vi "project 1.vi"() -> ()   [LabVIEW 2020]
uses:
  <vilib>/MakerHub/LINX/Public/Peripherals/Analog/Analog Read 1 Chan.vi
  <vilib>/MakerHub/LINX/Public/Peripherals/Analog/Analog Read N Chans.vi
  <vilib>/MakerHub/LINX/Private/Local IO/LinxAnalogRead.vi
  <vilib>/MakerHub/LINX/Public/Utilities/Check Channel.vi
  <vilib>/MakerHub/LINX/Public/Utilities/Open Serial.vi
  <vilib>/MakerHub/LINX/Public/Sensors/Motion/Servo/Servo Open One Channel.vi
  <vilib>/MakerHub/LINX/Private/Utilties/Generate Error.vi
  <vilib>/MakerHub/LINX/Public/Sensors/Motion/Servo/Servo Set Pulse Width One Channel.vi
  <vilib>/MakerHub/LINX/Public/Sensors/Motion/Servo/Servo Close One Channel.vi
  <vilib>/MakerHub/LINX/LMH-LINX.lvlib
  <vilib>/MakerHub/LINX/Public/Sensors/Motion/Servo/Servo.lvlib
panel:
  out "Angle":dbl=2.197357822357816
  out "Pulse width\nx+y":dbl=1024.4140625
  in  "stop":bool
  out "dv":dbl=0.1220703125
  out "Voltage 2":dbl=0.2099609375
  out "Voltage":dbl=0.33203125
  in  "Gain":dbl=200.0
  in  "Serial Port":refnum<visa-resource-name>="COM3"
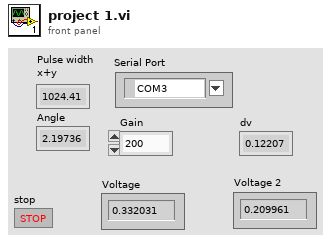
[diagram p1: front panel]
types:
  T1 = typedef "LMH-LINX.lvlib/LINX Ref.ctl" = cluster{"IO":T2, "Interface":T3, "LINX Device Config":T4}
  T2 = typedef "LMH-LINX.lvlib/Platform.ctl" = enum16{"Remote", "Local"}
  T3 = typedef "LMH-LINX.lvlib/Interface.ctl" = enum16{"Serial", "TCP"}
  T4 = typedef "LMH-LINX.lvlib/Device.lvlib/LINX Device Config.ctl" = cluster{"Interface":T3, "COM Port":refnum<visa-resource-name>, "TCP Configuration":T5, "Device Family":u8, "Device ID":u8, "Device Name":string, "TCP Ref":refnum<k5>, "Channels":T6}
  T5 = typedef "LMH-LINX.lvlib/Device.lvlib/TCP Config.ctl" = cluster{"IP Address":string, "Port":u16}
  T6 = typedef "LMH-LINX.lvlib/Channels.ctl" = cluster{"DI":u8[], "DO":u8[], "AI":u8[], "AO":u8[], "PWM":u8[], "QE":u8[], "UART":u8[], "I2C 2":u8[], "SPI":u8[], "CAN":u8[], "Servo":u8[], "AI Ref (V)":dbl, "AI Resolution (Bits)":u8, "AO Ref (V)":dbl, "AO Resolution (Bits)":u8}
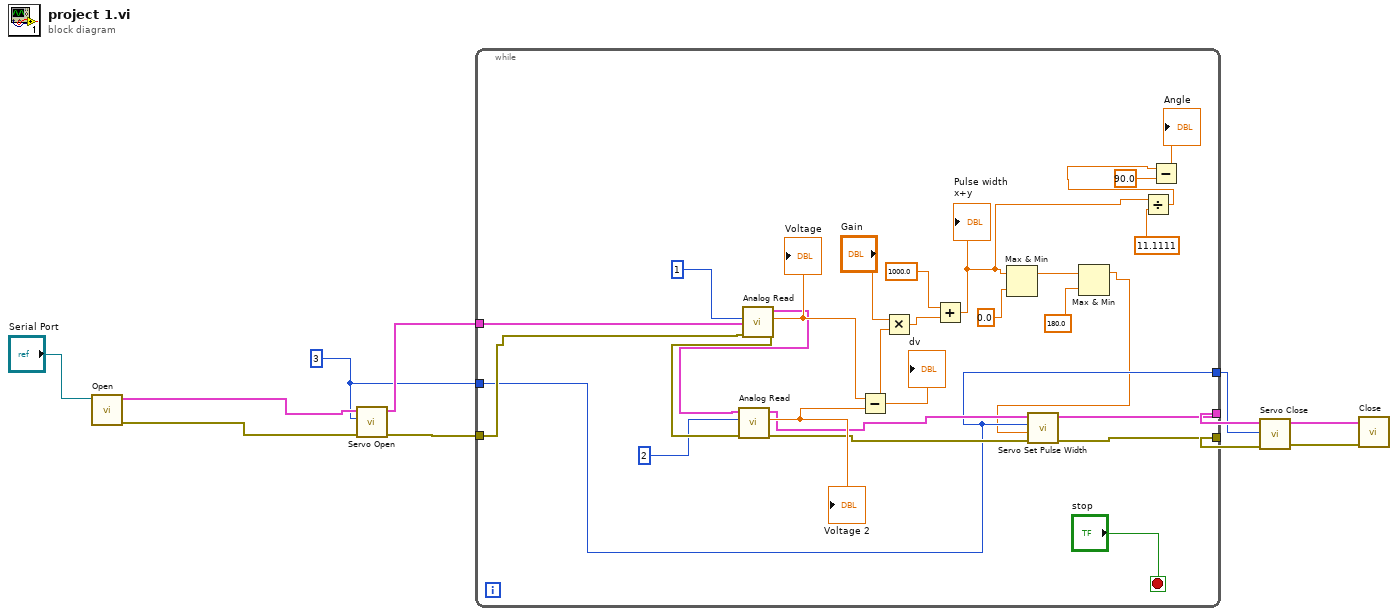
[diagram p0: block diagram]
diagram:
  w2 = u8 3 ("Servo Channel")
  n1 = call-poly <vilib>:"Open.vi"("Serial Port"="Serial Port") -> ("Error Out"=w10:errorcluster, "LINX Resource"=w6:T1)  [unwired: 8 in, 1 out]
  n2 = call-poly <vilib>:"Servo Open.vi"("Error In"=w10, "Servo Channel"=w2, "LINX Resource"=w6) -> ("Error Out"=w8:errorcluster, "LINX Resource"=w5:T1)  [unwired: 7 in]
  n3 = while {
    tunnel: w8 -> [w36]
    tunnel: [w33] -> w7
    tunnel: w5 -> [w29]
    tunnel: [w26] -> w4
    tunnel: w2 -> [w23]
    tunnel: [w23] -> w1
    stop <- "stop" stop-if-true
    n4 = call-poly <vilib>:"Analog Read.vi"("Error In"=w36, "Analog Channel"=u8 1, "LINX Resource"=w29) -> ("Error Out"=w35:errorcluster, "Voltage"=w37:dbl, "LINX Resource"=w28:T1)  [unwired: 5 in, 1 out]
    "Voltage" <- w37
    n5 = call-poly <vilib>:"Analog Read.vi"("Error In"=w35, "Analog Channel"=u8 2, "LINX Resource"=w28) -> ("Error Out"=w34:errorcluster, "Voltage"=w38:dbl, "LINX Resource"=w27:T1)  [unwired: 5 in, 1 out]
    "Voltage 2" <- w38
    n6 = Subtract(x=w37, y=w38) -> (x-y=w32:dbl)
    "dv" <- w32
    n7 = Multiply(x="Gain", y=w32) -> (x*y=w20:dbl)
    n8 = Add(x=1000.0, y=w20) -> (x+y=w12:dbl)
    "Pulse width\nx+y" <- w12
    n9 = Max & Min(x=w12, y=0.0) -> (max(x,y)=w19:dbl)  [unwired: 1 out]
    n10 = Max & Min(x=w19, y=180.0) -> (max(x,y)=w17:dbl)  [unwired: 1 out]
    n11 = call-poly <vilib>:"Servo Set Pulse Width.vi"("Error In"=w34, "Pulse Width (uS)"=w17, "Servo Channel"=w23, "LINX Resource"=w27) -> ("Error Out"=w33:errorcluster, "LINX Resource"=w26:T1)  [unwired: 6 in]
    n12 = Divide(x=w12, y=11.1111) -> (x/y=w15:dbl)
    n13 = Subtract(x=w15, y=90.0) -> (x-y=→"Angle":dbl)
  }
  n14 = call-poly <vilib>:"Servo Close.vi"("Error In"=w7, "Servo Channel"=w1, "LINX Resource"=w4) -> ("Error Out"=w9:errorcluster, "LINX Resource"=w3:T1)  [unwired: 7 in]
  n15 = call <vilib>:"Close.vi"("Error In"=w9, "LINX Resource"=w3) -> ()  [unwired: 9 in, 1 out]
